vi "Graph_Create.vi"(0 "reference":refnum<class "Graph.lvclass">, 5 "error in (no error)":errorcluster) -> (14 "reference out":refnum<class "Graph.lvclass">, 19 "error out":errorcluster)   [LabVIEW 2020, in "Graph.lvclass"]
uses:
  <resource>/Framework/Providers/Open_GDS/UML/Graph_class/Graph.lvclass
  <resource>/Framework/Providers/Open_GDS/UML/AbstractNode_class/AbstractNode.lvclass
  <resource>/Framework/Providers/Open_GDS/UML/AbstractEdge_class/AbstractEdge.lvclass
panel:
  # "The input reference should only\nbe wired when this method is called\nby a sub class constructor."
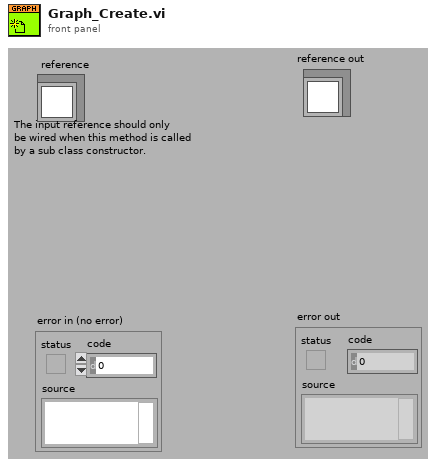
[diagram p1: front panel]
types:
  T1 = typedef "Graph.lvclass/ObjectAttributes.ctl" = cluster{"nodes":refnum<class "AbstractNode.lvclass">[], "edges":refnum<class "AbstractEdge.lvclass">[], "nodesToBeRemoved":refnum<class "AbstractNode.lvclass">[], "edgesToBeRemoved":refnum<class "AbstractEdge.lvclass">[], "needsLayout":bool, "LayoutNodes":refnum<class "AbstractNode.lvclass">[]}
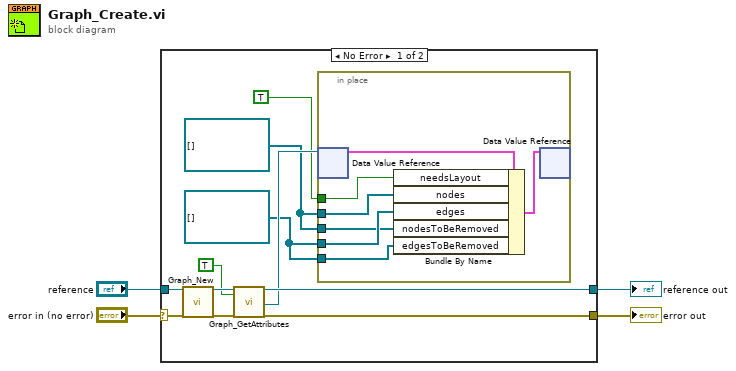
[diagram p0: block diagram]
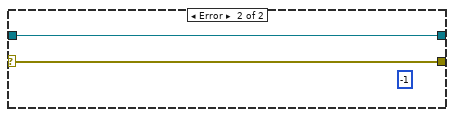
[diagram p2: hidden frame]
diagram:
  n1 = case shown="No Error" "error in (no error)" {
    selector: "error in (no error)" -> [w15 w24]
    tunnel: [w11 w23] -> w4
    tunnel: [w14 w24] -> w3
    tunnel: "reference" -> [w10 w23]
    frame No Error {
      w5 = refnum<class "AbstractEdge.lvclass">[] [] ("edges")
      w6 = refnum<class "AbstractNode.lvclass">[] [] ("nodes")
      n2 = call <resource>:"Graph_New.vi"("reference in"=w10, "error in (no error)"=w15) -> ("reference out"=w12:refnum<class "Graph.lvclass">, "error out"=w13:errorcluster)  [unwired: 2 in, 14 out]
      n3 = call <resource>:"Graph_GetAttributes.vi"("reference in"=w12, "OnlyGetDvrReference(False)"=TRUE, "error in (no error)"=w13) -> ("reference out"=w11:refnum<class "Graph.lvclass">, "DataRef"=w8:refnum<data-value>, "error out"=w14:errorcluster)  [unwired: 13 in, 1 out]
      n4 = in-place {
        in-place-border: TRUE ("needsLayout") -> [w21]
        in-place-border: w6 -> [w20]
        in-place-border: w5 -> [w19]
        in-place-border: w6 -> [w18]
        in-place-border: w5 -> [w17]
        n5 = in-place-dvr #1(w8) -> (w22:T1)  [unwired: 1 out]
        n6 = Bundle By Name(cluster=w22, "needsLayout"=w21, "nodes"=w20, "edges"=w19, "nodesToBeRemoved"=w18, "edgesToBeRemoved"=w17) -> (w16:T1)
        n7 = in-place-dvr #1(w16) -> ()  [unwired: 2 out]
      }
    }
    frame Error {
      (unwired) -1 ("Nr of open handles")
    }
  }
  "error out" <- w3
  "reference out" <- w4
